vi "BFS.vi"(7 "paths":i32[][][](array[numeric]), 9 "target":i32=4, 10 "processed states":set{i32[]}(c389)) -> (1 "result path":i32[][](array[numeric]))   [LabVIEW 2021]
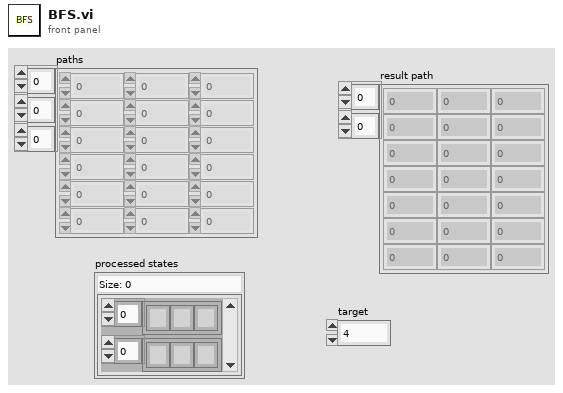
[diagram p1: front panel]
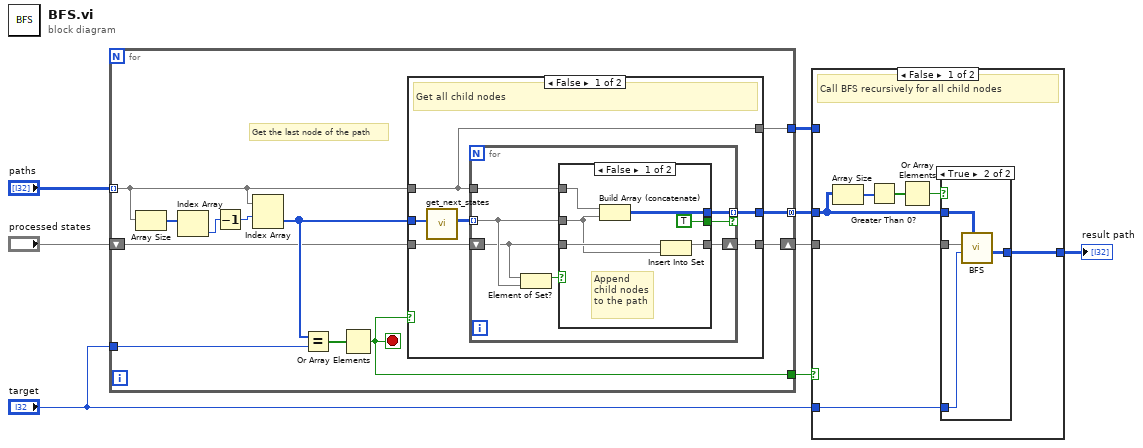
[diagram p0: block diagram]
diagram:
  n1 = for {
    tunnel: [w9] -> w8
    tunnel: "paths" -> [w16] mode=indexing
    tunnel: [w19] -> w6 mode=concatenating
    tunnel: [w18] -> w5
    shift-right: [w11] -> w2
    shift-left: "processed states" -> [w12]
    tunnel: "target" -> [w10]
    stop <- w9 stop-if-true
    # "Get the last node of the path"
    n2 = Array Size(array=w16) -> (size(s)=w15:i32[])
    n3 = Index Array(array=w15) -> (element=w14:i32)  [unwired: 1 in]
    n4 = Decrement(x=w14) -> (x-1=w13:i32)
    n5 = Index Array(array=w16, index (row)=w13) -> (element=w17:i32[])  [unwired: 1 in]
    n6 = Equal?(x=w17, y=w10) -> (x = y?=w20:bool[])
    n7 = Or Array Elements(Boolean array=w20) -> (logical OR=w9:bool)
    n8 = case shown="False" w9 {
      tunnel: w17 -> [w26 _]
      tunnel: w16 -> [w23 w42]
      tunnel: [w25 _] -> w19
      tunnel: [w23 w42] -> w18
      tunnel: w12 -> [w22 w41]
      tunnel: [w21 w41] -> w11
      frame False {
        # "Get all child nodes"
        n9 = call "get_next_states.vi"("state"=w26) -> ("next states"=w24:i32[][])  [unwired: 10 in]
        n10 = for {
          tunnel: w23 -> [w33]
          tunnel: [w32] -> w25 mode=indexing if=w27
          tunnel: w24 -> [w31] mode=indexing
          shift-right: [w28] -> w21
          shift-left: w22 -> [w29]
          n11 = Element of Set?(10:w31, 11:w29) -> (3:w30:bool)
          n12 = case shown="False" w30 {
            tunnel: w33 -> [w39 _]
            tunnel: [w38 _] -> w32
            tunnel: w31 -> [w36 _]
            tunnel: w29 -> [w37 w40]
            tunnel: [w35 w40] -> w28
            tunnel: [TRUE _] -> w27
            frame False {
              # "Append child nodes to the path"
              n13 = Build Array (concatenate)(w39, w36) -> (w38:i32[][])
              n14 = Insert Into Set(10:w36, 11:w37) -> (3:w35:set{i32[]})  [unwired: 1 out]
            }
            frame True {
            }
          }
        }
      }
      frame True {
      }
    }
  }
  n15 = case shown="False" w8 {
    tunnel: w6 -> [w45 _]
    tunnel: w5 -> [_ w54]
    tunnel: [w49 w54] -> w4
    tunnel: w2 -> [w44 _]
    tunnel: "target" -> [w43 _]
    frame False {
      # "Call BFS recursively for all child nodes"
      n16 = Array Size(array=w45) -> (size(s)=w48:i32[])
      n17 = Greater Than 0?(x=w48) -> (x > 0?=w47:bool[])
      n18 = Or Array Elements(Boolean array=w47) -> (logical OR=w46:bool)
      n19 = case shown="True" w46 {
        tunnel: [_ w53] -> w49
        tunnel: w45 -> [_ w52]
        tunnel: w44 -> [_ w51]
        tunnel: w43 -> [_ w50]
        frame False {
        }
        frame True {
          n20 = call "BFS.vi"("paths"=w52, "target"=w50, "processed states"=w51) -> ("result path"=w53:i32[][])  [unwired: 8 in]
        }
      }
    }
    frame True {
    }
  }
  "result path" <- w4
